vi "Scan Engine Custom FPGA Page - Local.vi"(8 "error in (no error)":errorcluster, 11 "Node Ptr":T1 format="%.0x") -> (0 "error out":errorcluster)   [LabVIEW 2020, in "SEECD System Explorer.lvlib"]
uses:
  SEECD System Explorer.lvlib
  <vilib>/NI VeriStand/Custom Device API/Custom Device API.lvlib
  Type Defs/FPGA Target.ctl
  <vilib>/NI VeriStand/Custom Device API/Custom Device Item Ref.ctl
panel:
  in  "SHDocVw.IWebBrowser2":refnum<k7>(container)
  out "Compilation Target":string
  out "FPGA Bitfile":path caption="Currently Loaded FPGA Personality"
  in  "Clear":bool
  in  "Bitfile Button":bool
  in  "Header":cluster{"Section Name":string}={"Section Name"="Local Chassis Custom FPGA Personality Settings"}
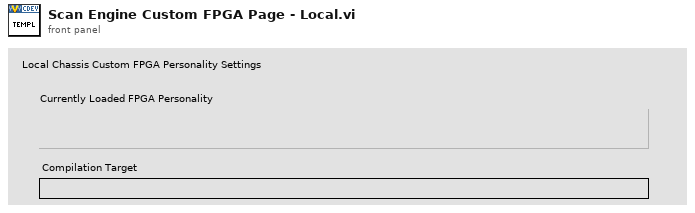
[diagram p1: front panel]
types:
  T1 = typedef "Custom Device API.lvlib/Custom Device Item Ref.ctl" = u64
  T2 = typedef "SEECD System Explorer.lvlib/FPGA Target.ctl" = enum16{"Local", "EtherCAT"}
  T3 = typedef "Custom Device API.lvlib/Custom Device Commands.ctl" = enum16{"Default", "Item renamed", "Shutdown", "Dynamic button pressed"}
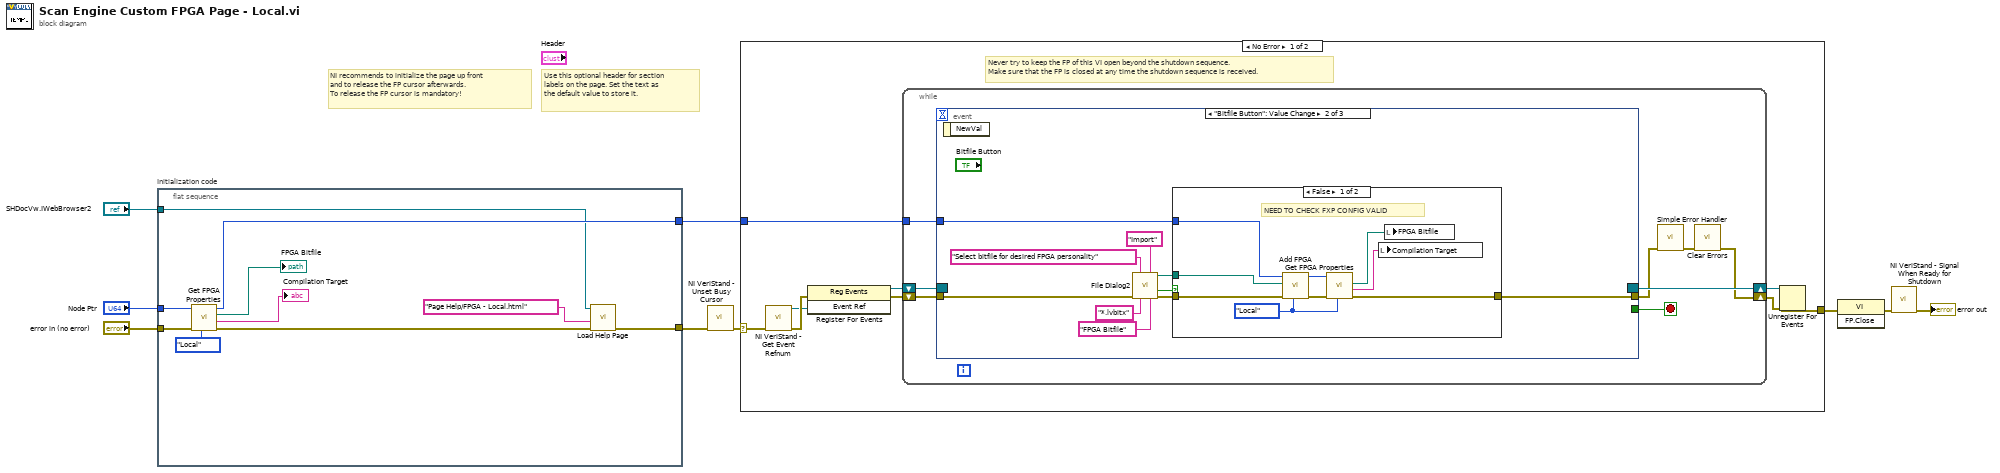
[diagram p0: block diagram]
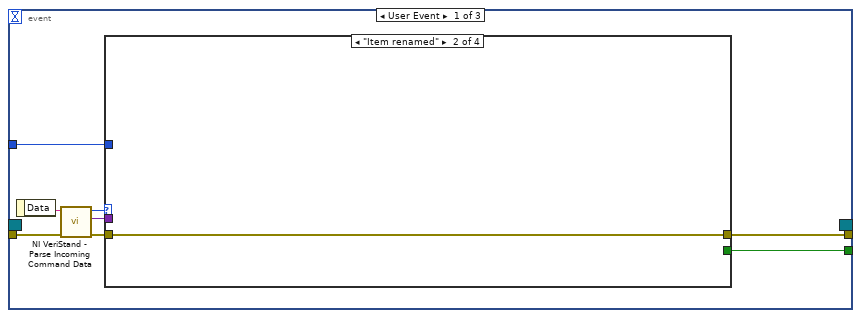
[diagram p2: hidden frame]
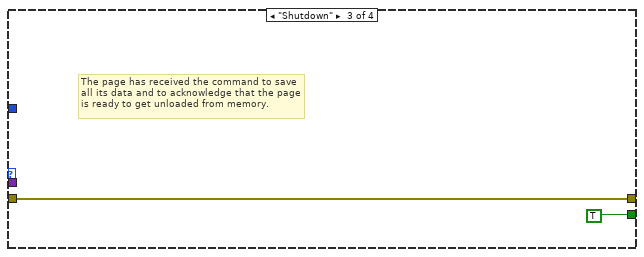
[diagram p4: hidden frame]
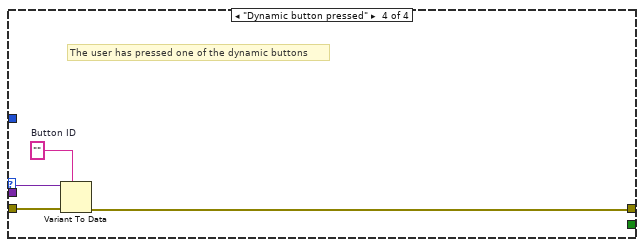
[diagram p5: hidden frame]
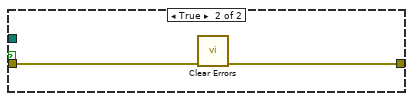
[diagram p6: hidden frame]
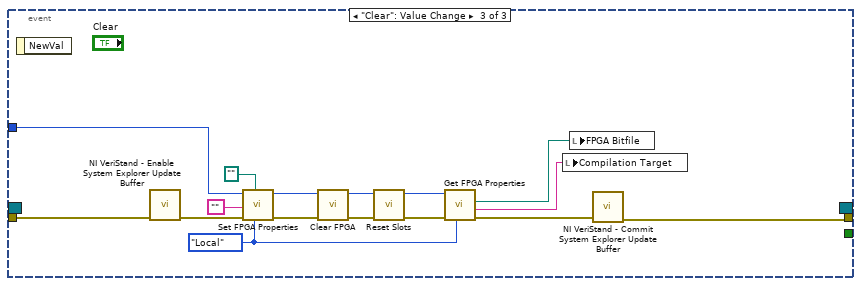
[diagram p7: hidden frame]
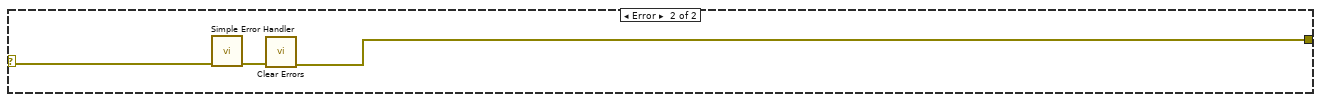
[diagram p8: hidden frame]
diagram:
  # "Use this optional header for section labels on the page. Set the text as the default value to store it."
  # "NI recommends to initialize the page up front\nand to release the FP cursor afterwards.\nTo release the FP cursor is mandatory!"
  n1 = flat-sequence "Initialization code" {
    tunnel: "error in (no error)" -> [w15]
    tunnel: "Node Ptr" -> [w16]
    tunnel: [w14] -> w3
    tunnel: "SHDocVw.IWebBrowser2" -> [w10]
    tunnel: [w11] -> w1
    frame #0 {
      n2 = call "Get FPGA Properties.vi"("FPGA Target"=FPGA_Target."Local", "error in (no error)"=w15, "Item Ref in"=w16) -> ("error out"=w12:errorcluster, "TargetClass"=→"Compilation Target":string, "Bitfile Path"=→"FPGA Bitfile":path, "Item Ref out"=w14:T1)  [unwired: 5 in]
      n3 = call "Load Help Page.vi"("error in (no error)"=w12, "HTML File to Load"="Page Help/FPGA - Local.html" ("name or relative path"), "Browser"=w10) -> ("error out"=w11:errorcluster)  [unwired: 8 in]
    }
  }
  n4 = call <vilib>:"NI VeriStand - Unset Busy Cursor.vi"("error in (no error)"=w1) -> ("error out"=w5:errorcluster)  [unwired: 10 out]
  n5 = case shown="No Error" w5 {
    selector: w5 -> [w20 w92]
    tunnel: [w25 w90] -> w9
    tunnel: w3 -> [w21 _]
    frame No Error {
      # "Never try to keep the FP of this VI open beyond the shutdown sequence.\nMake sure that the FP is closed at any time the shutdown sequence is received."
      n6 = call <vilib>:"NI VeriStand - Get Event Refnum.vi"("error in (no error)"=w20) -> ("error out"=w28:errorcluster, "Event Ref"=w24:refnum<user-event>)  [unwired: 9 out]
      n7 = register-events(error in=w28, w24) -> (reference out=w22:refnum<event-registration>, error out=w23:errorcluster)  [unwired: 1 in]
      n8 = while {
        tunnel: w21 -> [w32]
        shift-right: [w29] -> w26
        shift-left: w23 -> [w35]
        shift-right: [w36] -> w27
        shift-left: w22 -> [w34]
        stop <- w33 stop-if-true
        n9 = event shown="[1] \"Bitfile Button\": Value Change" {
          selector: w34 -> [_ _ _]
          dyn-events: [_ _ _] -> w36
          timeout: _ -> [_ _ _]
          tunnel: w35 -> [w44 w58 w79]
          tunnel: [w40 _ _] -> w33
          tunnel: [w39 w54 w78] -> w31
          tunnel: w32 -> [w38 w53 w86]
          event User Event {
            n10 = event-data() -> ("Data"=w43:string)  [unwired: 1 out]
            n11 = call <vilib>:"NI VeriStand - Parse Incoming Command Data.vi"("error in (no error)"=w44, "Incoming data"=w43) -> ("error out"=w42:errorcluster, "Outgoing data"=w37:variant, "Action"=w41:T3)  [unwired: 7 out]
            n12 = case shown="\"Item renamed\"" w41 {
              tunnel: w42 -> [w45 w46 w47 w52]
              tunnel: [_ _ TRUE _] -> w40
              tunnel: [w45 w46 w47 w49] -> w39
              tunnel: w38 -> [_ _ _ _]
              tunnel: w37 -> [_ _ _ w51]
              frame "Default", Default {
              }
              frame "Item renamed" {
              }
              frame "Shutdown" {
                # "The page has received the command to save all its data and to acknowledge that the page is ready to get unloaded from memory."
              }
              frame "Dynamic button pressed" {
                w50 = ""  # Button ID
                # "The user has pressed one of the dynamic buttons"
                n13 = Variant To Data(error in=w52, type=w50, Variant=w51) -> (error out=w49:errorcluster)  [unwired: 1 out]
              }
            }
          }
          event "Bitfile Button": Value Change {
            n14 = event-data() -> ()  [unwired: 2 out]
            n15 = call "File Dialog2"("prompt"="Select bitfile for desired FPGA personality", "button label"="Import", "error in"=w58, "pattern (all files)"="*.lvbitx", "pattern label"="FPGA Bitfile") -> ("selected path"=w55:path, "cancelled"=w57:bool, "error out"=w56:errorcluster)  [unwired: 7 in, 1 out]
            n16 = case shown="False" w57 {
              tunnel: w56 -> [w64 w73]
              tunnel: w55 -> [w70 _]
              tunnel: [w63 w72] -> w54
              tunnel: w53 -> [w71 _]
              frame False {
                w67 = FPGA_Target."Local" ("FPGA Target")
                # "NEED TO CHECK FXP CONFIG VALID"
                n17 = call "Add FPGA.vi"("FPGA Target"=w67, "error in (no error)"=w64, "Bitfile Path"=w70, "Item Ref in"=w71) -> ("error out"=w69:errorcluster, "Item Ref out"=w68:T1)  [unwired: 6 in]
                n18 = call "Get FPGA Properties.vi"("FPGA Target"=w67, "error in (no error)"=w69, "Item Ref in"=w68) -> ("error out"=w63:errorcluster, "TargetClass"=w65:string, "Bitfile Path"=w66:path)  [unwired: 5 in, 1 out]
                n19 = local write "Compilation Target"(w65) -> ()
                n20 = local write "FPGA Bitfile"(w66) -> ()
              }
              frame True {
                n21 = call <vilib>:"Clear Errors.vi"("error in (no error)"=w73) -> ("error out"=w72:errorcluster)  [unwired: 1 in, 5 out]
              }
            }
          }
          event "Clear": Value Change {
            w80 = FPGA_Target."Local" ("FPGA Target")
            n22 = event-data() -> ()  [unwired: 2 out]
            n23 = call <vilib>:"NI VeriStand - Enable System Explorer Update Buffer.vi"("error in (no error)"=w79) -> ("error out"=w87:errorcluster)  [unwired: 10 in]
            n24 = call "Set FPGA Properties.vi"("FPGA Target"=w80, "Bitfile Path"=path "", "error in (no error)"=w87, "TargetClass"="", "Item Ref in"=w86) -> ("error out"=w89:errorcluster, "Item Ref out"=w88:T1)  [unwired: 5 in]
            n25 = call "Clear FPGA.vi"("error in (no error)"=w89, "Item Ref in"=w88) -> ("error out"=w77:errorcluster, "Item Ref out"=w76:T1)  [unwired: 8 in]
            n26 = call "Reset Slots.vi"("error in (no error)"=w77, "Item Ref in"=w76) -> ("error out"=w74:errorcluster, "Item Ref out"=w75:T1)  [unwired: 8 in]
            n27 = call "Get FPGA Properties.vi"("FPGA Target"=w80, "error in (no error)"=w74, "Item Ref in"=w75) -> ("error out"=w81:errorcluster, "TargetClass"=w82:string, "Bitfile Path"=w83:path)  [unwired: 5 in, 1 out]
            n28 = local write "Compilation Target"(w82) -> ()
            n29 = local write "FPGA Bitfile"(w83) -> ()
            n30 = call <vilib>:"NI VeriStand - Commit System Explorer Update Buffer.vi"("error in (no error)"=w81) -> ("error out"=w78:errorcluster)  [unwired: 10 in]
          }
        }
        n31 = call <vilib>:"Simple Error Handler.vi"("error in (no error)"=w31) -> ("error out"=w30:errorcluster)  [unwired: 1 in, 7 out]
        n32 = call <vilib>:"Clear Errors.vi"("error in (no error)"=w30) -> ("error out"=w29:errorcluster)  [unwired: 1 in, 5 out]
      }
      n33 = Unregister For Events(event registration refnum=w27, error in=w26) -> (error out=w25:errorcluster)
    }
    frame Error {
      n34 = call <vilib>:"Simple Error Handler.vi"("error in (no error)"=w92) -> ("error out"=w91:errorcluster)  [unwired: 1 in, 7 out]
      n35 = call <vilib>:"Clear Errors.vi"("error in (no error)"=w91) -> ("error out"=w90:errorcluster)  [unwired: 1 in, 5 out]
    }
  }
  n36 = invoke class="VI" method="FP.Close"(error in=w9) -> (error out=w8:errorcluster)  [unwired: 2 in, 2 out]
  n37 = call <vilib>:"NI VeriStand - Signal When Ready for Shutdown.vi"("error in (no error)"=w8) -> ("error out"=→"error out":errorcluster)  [unwired: 10 out]
